vi "FindBin.vi"(0 "Threshold":dbl=10.0, 2 "NXT/EV3 IN":T2, 3 "Port":T1 items=["Port 1", "Port 2", "Port 3", "Port 4"]) -> (1 "Out":bool, 4 "NXT/EV3 OUT":T2)   [LabVIEW 2016, in "13.03 Robot.lvrbt"]
uses:
  13.03 Robot.lvrbt
  <vilib>/NXT/Subs/LVHSConnector.ctl
  <vilib>/NXT/LegoClasses/BrickReference/BrickReference.lvclass
  <vilib>/NXT/Block Support/NXT_InputPort.ctl
  <vilib>/NXT/Dual Mode Library/Sensors/EV3_Ultrasonic_CM.vi
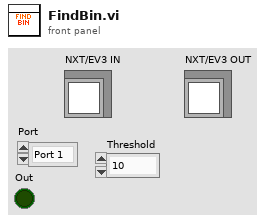
[diagram p1: front panel]
types:
  T1 = typedef "NXT_InputPort.ctl" = u32
  T2 = typedef "LVHSConnector.ctl" = refnum<class "BrickReference.lvclass">
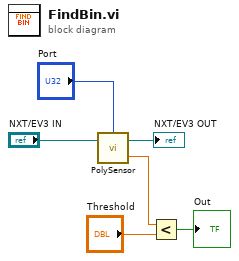
[diagram p0: block diagram]
diagram:
  n1 = call-poly <vilib>:"PolySensor.vi"("NXT/EV3"="NXT/EV3 IN", "Port (Port 1)"="Port") -> ("Centimeters"=w3:sgl, "NXT/EV3"=→"NXT/EV3 OUT":T2)  [unwired: 1 in]
  n2 = Less?(x=w3, y="Threshold") -> (x < y?=→"Out":bool)
